vi "Bits2Bools.vi"(4 "Bits":string) -> (1 "Bools":bool[](array[boolean]))   [LabVIEW 2025]
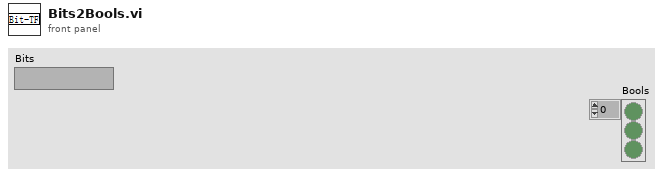
[diagram p1: front panel]
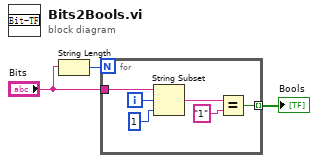
[diagram p0: block diagram]
diagram:
  n1 = String Length(string="Bits") -> (length=w3:i32)
  n2 = for {
    N: w3 -> [_]
    tunnel: "Bits" -> [w8]
    tunnel: [w4] -> w1 mode=indexing
    i -> [w9]
    n3 = String Subset(string=w8, offset (0)=w9, length (rest)=1 ("长度（剩余）")) -> (substring=w6:string)
    n4 = Equal?(x=w6, y="1") -> (x = y?=w4:bool)
  }
  "Bools" <- w1
